vi "VIH Project Tree - Get Tree Item Tags.vi"(8 "error in":errorcluster, 9 "Recursively (T)":bool=TRUE, 10 "Parent Item Tag":string, 11 "Project Tree":T1) -> (0 "error out":errorcluster, 1 "Child Item Tags":string[](array[string]), 2 "dup Parent Item Tag":string, 3 "dup Project Tree":T1)   [LabVIEW 2014]
doc: "::: VI Helpeks :::\nCopyright (c) 2000-2026 Konstantin Shifershteyn. All rights reserved."
uses:
  VIH Project Tree Typedef - Tree Refnum.ctl
panel:
  # "VI Helpeks\nCopyright (c) 2012-2026 Konstantin Shifershteyn"
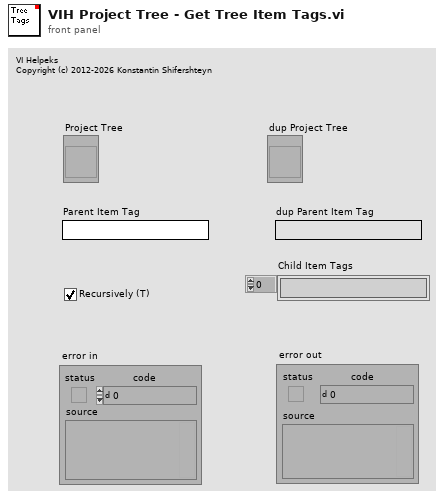
[diagram p1: front panel]
types:
  T1 = typedef "VIH Project Tree Typedef - Tree Refnum.ctl" = refnum<vi>
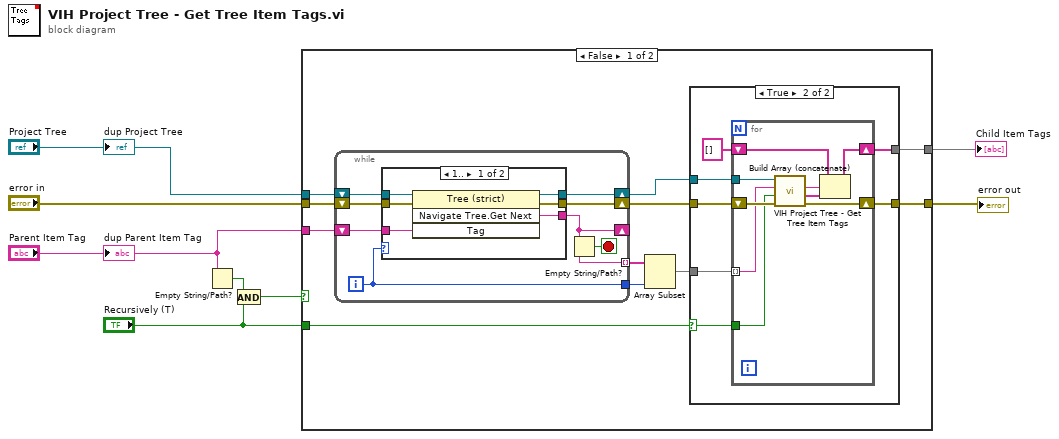
[diagram p0: block diagram]
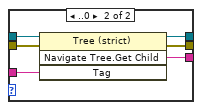
[diagram p3: hidden frame]
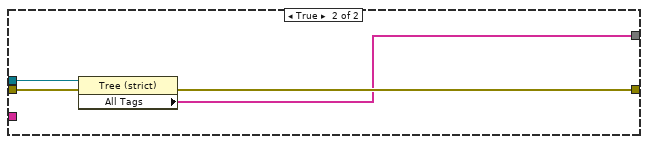
[diagram p4: hidden frame]
diagram:
  n1 = Empty String/Path?(string/path="Parent Item Tag") -> (empty?=w6:bool)
  n2 = And(x=w6, y="Recursively (T)") -> (x .and. y?=w5:bool)
  n3 = case shown="False" w5 {
    tunnel: "Project Tree" -> [w17 w61]
    tunnel: "error in" -> [w16 w60]
    tunnel: "Parent Item Tag" -> [w15 _]
    tunnel: [w10 w59] -> w4
    tunnel: [w9 w58] -> w1
    tunnel: "Recursively (T)" -> [w13 _]
    frame False {
      n4 = while {
        shift-right: [w43] -> _
        shift-left: w15 -> [w45]
        tunnel: [w43] -> w19 mode=indexing
        tunnel: [w42] -> w18
        shift-right: [w41] -> w14
        shift-left: w17 -> [w39]
        shift-right: [w40] -> w12
        shift-left: w16 -> [w38]
        i -> [w42]
        stop <- w44 stop-if-true
        n5 = case shown="1.." w42 {
          tunnel: w45 -> [w46 w57]
          tunnel: [w51 w56] -> w43
          tunnel: [w50 w55] -> w41
          tunnel: [w49 w54] -> w40
          tunnel: w39 -> [w48 w53]
          tunnel: w38 -> [w47 w52]
          frame 1.. {
            n6 = invoke class="Tree (strict)" method="Navigate Tree.Get Next"(reference=w48, error in=w47, "Tag"=w46) -> (reference out=w50:T1, error out=w49:errorcluster, "Navigate Tree:Get Next Item"=w51:string)  [unwired: 1 in, 1 out]
          }
          frame ..0 {
            n7 = invoke class="Tree (strict)" method="Navigate Tree.Get Child"(reference=w53, error in=w52, "Tag"=w57) -> (reference out=w55:T1, error out=w54:errorcluster, "Navigate Tree:Get Child"=w56:string)  [unwired: 1 in, 1 out]
          }
        }
        n8 = Empty String/Path?(string/path=w43) -> (empty?=w44:bool)
      }
      n9 = Array Subset(array=w19, length=w18) -> (w11:string[])  [unwired: 1 in]
      n10 = case shown="True" w13 {
        selector: w13 -> [_ w22]
        tunnel: w14 -> [_ w28]
        tunnel: w12 -> [w20 w27]
        tunnel: w11 -> [w21 w26]
        tunnel: [w20 w25] -> w10
        tunnel: [w21 w24] -> w9
        frame False {
        }
        frame True {
          n11 = for {
            tunnel: w28 -> [w37]
            shift-right: [w35] -> w25
            shift-left: w27 -> [w36]
            tunnel: w26 -> [w34] mode=indexing
            shift-right: [w30] -> w24
            shift-left: string[] [] -> [w31]
            tunnel: w22 -> [w29]
            n12 = call "VIH Project Tree - Get Tree Item Tags.vi"("error in"=w36, "Recursively (T)"=w29, "Parent Item Tag"=w34, "Project Tree"=w37) -> ("error out"=w35:errorcluster, "Child Item Tags"=w32:string[], "dup Parent Item Tag"=w33:string)  [unwired: 4 in, 1 out]
            n13 = Build Array (concatenate)(w31, w33, w32) -> (w30:string[])
          }
        }
      }
    }
    frame True {
      n14 = property class="Tree (strict)"(reference=w61, error in=w60) -> (error out=w59:errorcluster, "All Tags"=w58:string[])  [unwired: 1 out]
    }
  }
  "error out" <- w4
  "Child Item Tags" <- w1
  "dup Project Tree" <- "Project Tree"
  "dup Parent Item Tag" <- "Parent Item Tag"
